vi "Save QD suggestions.vi"(8 "error in":errorcluster, 10 "Position":T1, 11 "Suggestions":cluster{"Class Name":string, "Count":i32}[](array[cluster])) -> (0 "error out":errorcluster)   [LabVIEW 2020]
uses:
  QD Suggestion.ctl
  QD Data.ctl
  <vilib>/Utility/miscctls.llb/LVPositionTypeDef.ctl
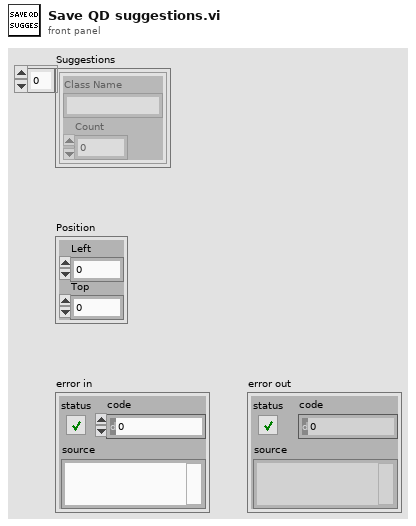
[diagram p1: front panel]
types:
  T1 = typedef "LVPositionTypeDef.ctl" = cluster{"Left":i32, "Top":i32}
  T2 = typedef "QD Data.ctl" = cluster{T3[], cluster{"Left":i32, "Top":i32}}
  T3 = typedef "QD Suggestion.ctl" = cluster{"Data":string, "qd":string[], "Type":string}
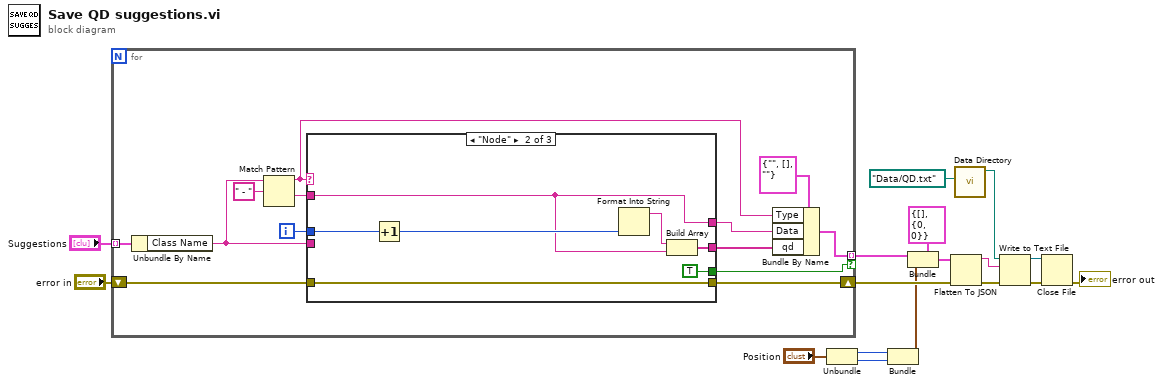
[diagram p0: block diagram]
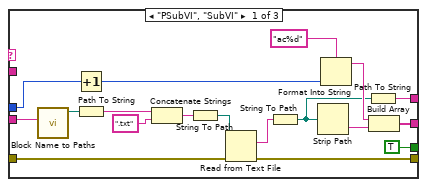
[diagram p2: hidden frame]
diagram:
  n1 = for {
    tunnel: "Suggestions" -> [w30] mode=indexing
    tunnel: [w28] -> w9 mode=indexing if=w25
    shift-right: [w21] -> w11
    shift-left: "error in" -> [w22]
    i -> [w26]
    n2 = Unbundle By Name(w30) -> ("Class Name"=w20:string)
    n3 = Match Pattern(string=w20, regular expression=" - " ("search string/char (-)")) -> (before substring=w19:string, after substring=w18:string)  [unwired: 1 in, 2 out]
    n4 = case shown="\"Node\"" w19 {
      tunnel: [TRUE ("Boolean") TRUE ("Boolean") _] -> w25
      tunnel: w18 -> [_ w49 _]
      tunnel: w20 -> [w43 _ _]
      tunnel: [w36 w52 _] -> w27
      tunnel: w26 -> [w35 w51 _]
      tunnel: [w34 w49 _] -> w24
      tunnel: w22 -> [w33 w50 w56]
      tunnel: [w32 w50 w56] -> w21
      frame "PSubVI", "SubVI" {
        n5 = call "Block Name to Paths.vi"("Block Name"=w43) -> ("Block Path"=w44:path)  [unwired: 9 in, 1 out]
        n6 = Increment(x=w35) -> (x+1=w40:i32)
        n7 = Path To String(path=w44) -> (string=w48:string)
        n8 = Concatenate Strings(w48, ".txt" ("string")) -> (w46:string)
        n9 = String To Path(string=w46) -> (path=w42:path)
        n10 = Read from Text File(file (use dialog)=w42, error in=w33) -> (text=w45:string, error out=w32:errorcluster)  [unwired: 2 in, 2 out]
        n11 = String To Path(string=w45) -> (path=w31:path)
        n12 = Strip Path(path=w31) -> (name=w37:string)  [unwired: 1 out]
        n13 = Format Into String(format string="ac%d", w40) -> (resulting string=w38:string)  [unwired: 2 in, 1 out]
        n14 = Path To String(path=w31) -> (string=w34:string)
        n15 = Build Array(w38, w37) -> (w36:string[])
      }
      frame "Node" {
        n16 = Increment(x=w51) -> (x+1=w54:i32)
        n17 = Format Into String(w54) -> (resulting string=w53:string)  [unwired: 3 in, 1 out]
        n18 = Build Array(w53, w49) -> (w52:string[])
      }
      frame Default {
      }
    }
    n19 = Bundle By Name(cluster=T3 {"Data"="", "qd"=[], "Type"=""}, "Type"=w19, "Data"=w24, "qd"=w27) -> (w28:T3)
  }
  n20 = Unbundle("Position") -> ("Left"=w7:i32, "Top"=w6:i32)
  n21 = Bundle("Left"=w7, "Top"=w6) -> (w5:cluster{"Left":i32, "Top":i32})  [unwired: 1 in]
  n22 = Bundle(cluster=T2 {[], {"Left"=0, "Top"=0}}, w9, w5) -> (w4:T2)
  n23 = Flatten To JSON(anything=w4, error in (no error)=w11) -> (JSON string=w15:string, 11:w16:errorcluster)  [unwired: 1 in]
  n24 = call "Data Directory.vi"("Subdirectory"=path "Data/QD.txt" ("file (use dialog)")) -> ("Data directory"=w1:path)  [unwired: 9 in, 1 out]
  n25 = Write to Text File(file (use dialog)=w1, text=w15, error in=w16) -> (refnum out=w14:refnum<file>, error out=w13:errorcluster)  [unwired: 1 in, 1 out]
  n26 = Close File(refnum=w14, error in=w13) -> (error out=→"error out":errorcluster)  [unwired: 1 out]
